vi "Cond B Cond First.vi"(8 "error in":errorcluster) -> (0 "error out":errorcluster, 1 "Result":i32)   [LabVIEW 2026]
doc: "Conditional Disable repro: each frame returns its own index."
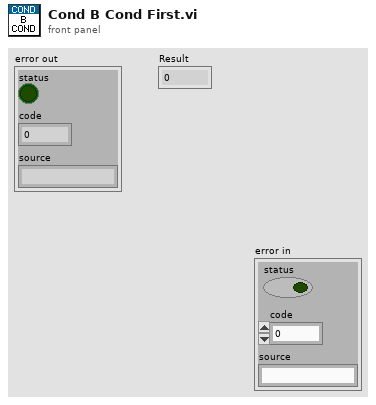
[diagram p1: front panel]
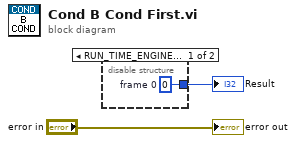
[diagram p0: block diagram]
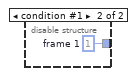
[diagram p2: hidden frame]
diagram:
  n1 = disable-structure shown="RUN_TIME_ENGINE==False" {
    disable-tunnel: [w3 w4] -> w2
    frame condition #0 (active) {
      w3 = 0  # frame 0
    }
    frame condition #1 {
      w4 = 1  # frame 1
    }
  }
  "Result" <- w2
  "error out" <- "error in"
